vi "MQTT Reason - Disconnect Type (DEVELOPER).vi"() -> ()   [LabVIEW 2019, in "KoRE-MQTT.lvlib"]
doc: "Copyright (c) 2025 KoRElibs.com\nSPDX-License-Identifier: EUPL-1.2\n\nThis VI is licensed under the European Union Public License (EUPL) Version 1.2. You may use this VI unmodified in proprietary works. If you distribute a modified version of this file, the modified file must be released under the EUPL-1.2. Full license: https://joinup.ec.europa.eu/asset/eupl/eupl/1.2/"
uses:
  KoRE-MQTT.lvlib
  MQTT Reason - Disconnect Type.ctl
panel:
  out "Disconnect Reason String":string
  in  "Disconnect Reason Code":T1 items=[" Close the connection normally. Do not send the Will Message."=0, " The Client wishes to disconnect but requires that the Server also publishes its Will Message."=4, " The Connection is closed but the sender either does not wish to reveal the reason, or none of the other Reason Codes apply."=128, " The received packet does not conform to this specification."=129, " An unexpected or out of order packet was received."=130, " The packet received is valid but cannot be processed by this implementation."=131, " The request is not authorized."=135, " The Server is busy and cannot continue processing requests from this Client."=137, " The Server is shutting down."=139, " The Connection is closed because no packet has been received for 1.5 times the Keepalive time."=141, " Another Connection using the same ClientID has connected causing this Connection to be closed."=142, " The Topic Filter is correctly formed, but is not accepted by this Server."=143, " The Topic Name is correctly formed, but is not accepted by this Client or Server."=144, " The Client or Server has received more than Receive Maximum publication for which it has not sent PUBACK or PUBCOMP."=147, " The Client or Server has received a PUBLISH packet containing a Topic Alias which is greater than the Maximum Topic Alias it sent in the CONNECT or CONNACK packet."=148, " The packet size is greater than Maximum Packet Size for this Client or Server."=149, " The received data rate is too high."=150, " An implementation or administrative imposed limit has been exceeded."=151, " The Connection is closed due to an administrative action."=152, " The payload format does not match the one specified by the Payload Format Indicator."=153, " The Server has does not support retained messages."=154, " The Client specified a QoS greater than the QoS specified in a Maximum QoS in the CONNACK."=155, " The Client should temporarily change its Server."=156, " The Server is moved and the Client should permanently change its server location."=157, " The Server does not support Shared Subscriptions."=158, " This connection is closed because the connection rate is too high."=159, " The maximum connection time authorized for this connection has been exceeded."=160, " The Server does not support Subscription Identifiers; the subscription is not accepted."=161, " The Server does not support Wildcard Subscriptions; the subscription is not accepted."=162]
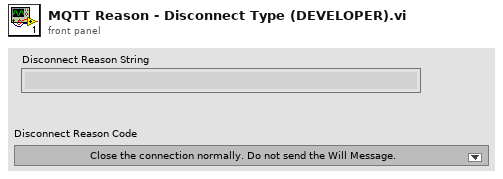
[diagram p1: front panel]
types:
  T1 = typedef "KoRE-MQTT.lvlib/MQTT Reason - Disconnect Type.ctl" = u16
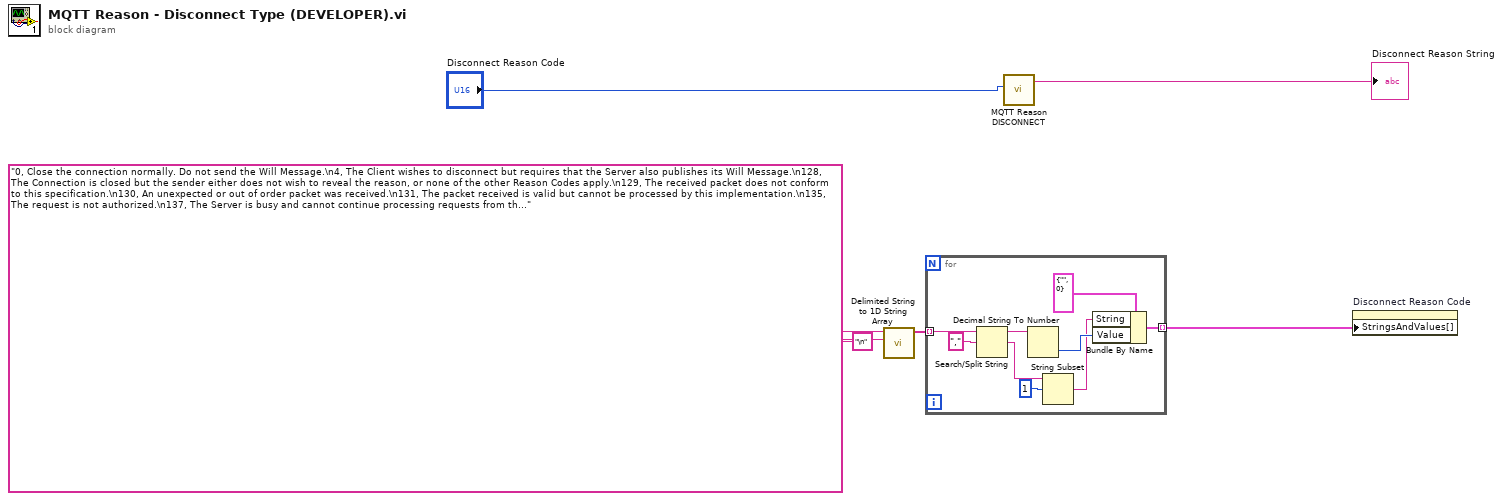
[diagram p0: block diagram]
diagram:
  n1 = call <vilib>:"Delimited String to 1D String Array.vi"("delimiter"="\n", "delimited string"="0, Close the connection normally. Do not send the Will Message.\n4, The Client wishes to disconnect but requires that the Server also publishes its Will Message.\n128, The Connection is closed but the sender either does not wish to reveal the reason, or none of the other Reason Codes apply.\n129, The received packet does not conform to this specification.\n130, An unexpected or out of order packet was received.\n131, The packet received is valid but cannot be processed by this implementation.\n135, The request is not authorized.\n137, The Server is busy and cannot continue processing requests from this Client.\n139, The Server is shutting down.\n141, The Connection is closed because no packet has been received for 1.5 times the Keepalive time.\n142, Another Connection using the same ClientID has connected causing this Connection to be closed.\n143, The Topic Filter is correctly formed, but is not accepted by this Server.\n144, The Topic Name is correctly formed, but is not accepted by this Client or Server.\n147, The Client or Server has received more than Receive Maximum publication for which it has not sent PUBACK or PUBCOMP.\n148, The Client or Server has received a PUBLISH packet containing a Topic Alias which is greater than the Maximum Topic Alias it sent in the CONNECT or CONNACK packet.\n149, The packet size is greater than Maximum Packet Size for this Client or Server.\n150, The received data rate is too high.\n151, An implementation or administrative imposed limit has been exceeded.\n152, The Connection is closed due to an administrative action.\n153, The payload format does not match the one specified by the Payload Format Indicator.\n154, The Server has does not support retained messages.\n155, The Client specified a QoS greater than the QoS specified in a Maximum QoS in the CONNACK.\n156, The Client should temporarily change its Server.\n157, The Server is moved and the Client should permanently change its server location.\n158, The Server does not support Shared Subscriptions.\n159, This connection is closed because the connection rate is too high.\n160, The maximum connection time authorized for this connection has been exceeded.\n161, The Server does not support Subscription Identifiers; the subscription is not accepted.\n162, The Server does not support Wildcard Subscriptions; the subscription is not accepted." ("spreadsheet string")) -> ("string array"=w4:string[])  [unwired: 9 in]
  n2 = for {
    tunnel: w4 -> [w15] mode=indexing
    tunnel: [w7] -> w3 mode=indexing
    n3 = Search/Split String(string=w15, search string/char (-)=",") -> (substring before match=w13:string, match + rest of string=w12:string)  [unwired: 1 in, 1 out]
    n4 = Decimal String To Number(string=w13) -> (number=w9:i32)  [unwired: 2 in, 1 out]
    n5 = String Subset(string=w12, offset (0)=1) -> (substring=w8:string)  [unwired: 1 in]
    n6 = Bundle By Name(cluster=cluster{"String":string, "Value":u16} {"String"="", "Value"=0}, "String"=w8, "Value"=w9) -> (w7:cluster{"String":string, "Value":u16})
  }
  n7 = call "MQTT Reason DISCONNECT.vi"("Disconnect Reason Code"="Disconnect Reason Code") -> ("String"=→"Disconnect Reason String":string)  [unwired: 10 in]
  n8 = property on="Disconnect Reason Code" class="Ring (strict)"("StringsAndValues[]"=w3) -> ()  [unwired: 2 in, 2 out]
